vi "Restart.CacheCurrentLocation.vi"(8 "error in (no error)":errorcluster, 10 "Result":T1, 11 "State Variables":T2={"NIVS.BaseLogPath"=path "", "NIVS.SystemDefinitionFile"=path "", "NIVS.Events"={"SequenceEvent"=refnum, "SystemChangeEvent"=refnum, "WorkspaceEvent"=refnum}, "NIVS.SequenceState"=enum."Idle", "NIVS.GatewayIPAddress"="", "NIVS.DataLogSpecRef"=refnum, "NIVS.DataLogManagerRef"=refnum, "NIVS.LogSessionGUID"="", "NIVS.WorkspaceManager"=refnum, "NIVS.Deployed"=FALSE, "NIVS.ProfileRef"=refnum, "NIVS.ProfileCallback"=refnum, "NIVS.SystemStateRefs"={"CustDatRef"=refnum, "EvtRef"=refnum, "Target State User Event"=refnum}, "UI.Abort"=refnum, "UI.Pause"=refnum, "UI.EnableLogging"=refnum, "UI.Start"=refnum, "UI.LogChannels"=refnum, "UI.StartIteration"=refnum, "UI.StartStep"=refnum, "UI.Sequence"=refnum, "UI.PreviewMode"=refnum, "UI.Graph"=refnum, "UI.BaseFileName"=refnum, "UI.Profiles"=refnum, "UI.CurrentStep"=refnum, "UI.CurrentIteration"=refnum, "UI.TotalIterations"=refnum, "Sequence.AbortChannel"="", "Sequence.StepInfoChannel"="", "Sequence.Iterations"=0, "Sequence.IterationInfoChannel"="", "Sequence.#ofColumns"=0, "Events.State"=refnum, "Events.Test Result"=refnum, "Events.Progress"=refnum, "INI.Settings"={"Build Location"=path "C:/Simple Sequence Editor/SequenceRepo", "LoggingLocation"=path ""}, "UI.Skip"=refnum, "Sequence.SkipChannel"="", "Restart.Path"=path "", "UI.Duration"=refnum, "Sequence.DurationChannel"=""}) -> (0 "error out":errorcluster, 2 "Restart?":bool, 3 "State Variables out":T2={"NIVS.BaseLogPath"=path "", "NIVS.SystemDefinitionFile"=path "", "NIVS.Events"={"SequenceEvent"=refnum, "SystemChangeEvent"=refnum, "WorkspaceEvent"=refnum}, "NIVS.SequenceState"=enum."Idle", "NIVS.GatewayIPAddress"="", "NIVS.DataLogSpecRef"=refnum, "NIVS.DataLogManagerRef"=refnum, "NIVS.LogSessionGUID"="", "NIVS.WorkspaceManager"=refnum, "NIVS.Deployed"=FALSE, "NIVS.ProfileRef"=refnum, "NIVS.ProfileCallback"=refnum, "NIVS.SystemStateRefs"={"CustDatRef"=refnum, "EvtRef"=refnum, "Target State User Event"=refnum}, "UI.Abort"=refnum, "UI.Pause"=refnum, "UI.EnableLogging"=refnum, "UI.Start"=refnum, "UI.LogChannels"=refnum, "UI.StartIteration"=refnum, "UI.StartStep"=refnum, "UI.Sequence"=refnum, "UI.PreviewMode"=refnum, "UI.Graph"=refnum, "UI.BaseFileName"=refnum, "UI.Profiles"=refnum, "UI.CurrentStep"=refnum, "UI.CurrentIteration"=refnum, "UI.TotalIterations"=refnum, "Sequence.AbortChannel"="", "Sequence.StepInfoChannel"="", "Sequence.Iterations"=0, "Sequence.IterationInfoChannel"="", "Sequence.#ofColumns"=0, "Events.State"=refnum, "Events.Test Result"=refnum, "Events.Progress"=refnum, "INI.Settings"={"Build Location"=path "C:/Simple Sequence Editor/SequenceRepo", "LoggingLocation"=path ""}, "UI.Skip"=refnum, "Sequence.SkipChannel"="", "Restart.Path"=path "", "UI.Duration"=refnum, "Sequence.DurationChannel"=""})   [LabVIEW 2015, in "Simple Sequence Tools - Execution.lvlib"]
uses:
  Simple Sequence Tools - Execution.lvlib
  Types/Main.StateVariables.ctl
  Types/Execute.UserEventRefs.ctl
  <vilib>/NI Veristand/Execution/Workspace/SystemStateRegEventRef.ctl
  <vilib>/NI Veristand/Execution/Workspace/Target State Info.ctl
  <vilib>/NI Veristand/Execution/Workspace/Target State.ctl
  Types/Execution.SequenceState.ctl
  <vilib>/NI Veristand/Execution/DataLogging/DataLoggingSpecification Ref.ctl
  NationalInstruments.VeriStand.ClientAPI
  <vilib>/NI Veristand/Execution/DataLogging/IDataLogging Ref.ctl
  <vilib>/NI Veristand/Execution/Workspace/WorkspaceAPI.ctl
  NationalInstruments.VeriStand.RealTimeSequenceDefinitionApi
  <vilib>/NI Veristand/Execution/Workspace/SystemStateEventRef.ctl
  Shared/Types/INI.Settings.ctl
  Types/Results.Value.ctl
  <vilib>/NI Veristand/Execution/Workspace/NI VeriStand - Get Single Channel Value.vi
  <vilib>/NI Veristand/Execution/Workspace/NI_VS Workspace ExecutionAPI.lvlib
  <vilib>/NI Veristand/Execution/DataLogging/NI_VS Data Logging API.lvlib
  Shared/Simple Sequence Tools - Shared.lvlib
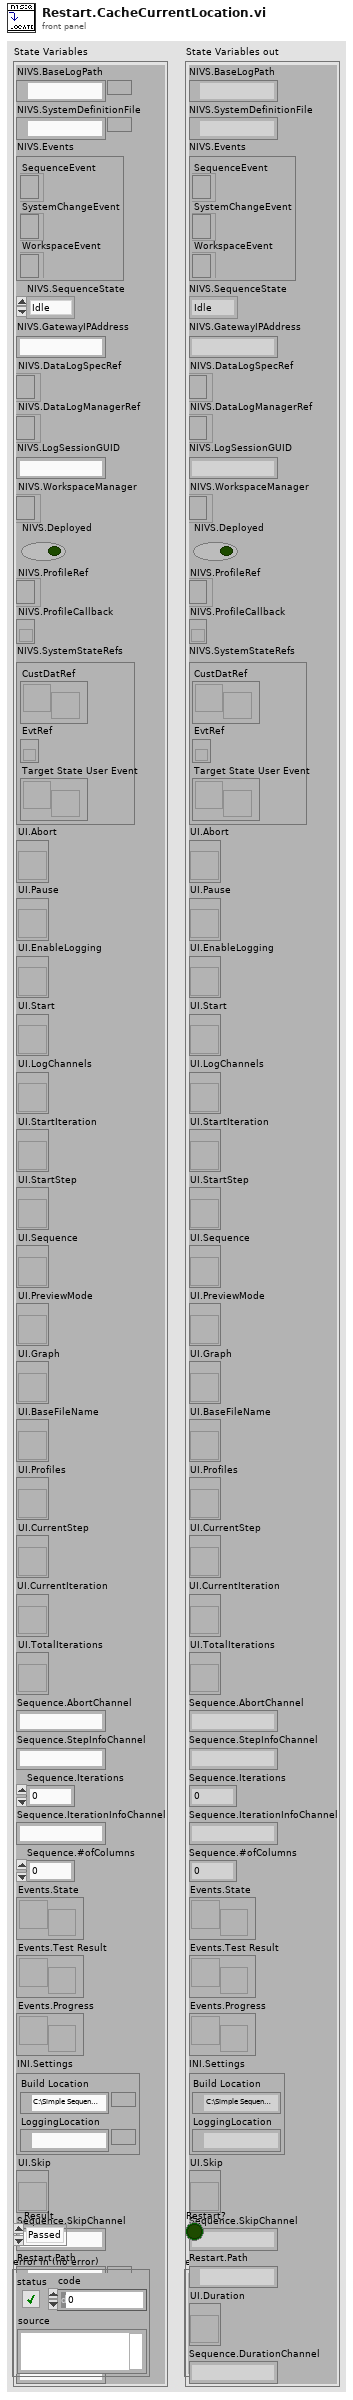
[diagram p1: front panel]
types:
  T1 = typedef "Simple Sequence Tools - Execution.lvlib/Results.Value.ctl" = enum8{"Passed", "Failed", "Aborted"}
  T2 = typedef "Simple Sequence Tools - Execution.lvlib/Main.StateVariables.ctl" = cluster{"NIVS.BaseLogPath":path, "NIVS.SystemDefinitionFile":path, "NIVS.Events":T3, "NIVS.SequenceState":T5, "NIVS.GatewayIPAddress":string, "NIVS.DataLogSpecRef":T6, "NIVS.DataLogManagerRef":T7, "NIVS.LogSessionGUID":string, "NIVS.WorkspaceManager":T8, "NIVS.Deployed":bool, "NIVS.ProfileRef":refnum<k24>, "NIVS.ProfileCallback":refnum<k27>, "NIVS.SystemStateRefs":T9, "UI.Abort":refnum<vi>, "UI.Pause":refnum<vi>, "UI.EnableLogging":refnum<vi>, "UI.Start":refnum<vi>, "UI.LogChannels":refnum<vi>, "UI.StartIteration":refnum<vi>, "UI.StartStep":refnum<vi>, "UI.Sequence":refnum<vi>, "UI.PreviewMode":refnum<vi>, "UI.Graph":refnum<vi>, "UI.BaseFileName":refnum<vi>, "UI.Profiles":refnum<vi>, "UI.CurrentStep":refnum<vi>, "UI.CurrentIteration":refnum<vi>, "UI.TotalIterations":refnum<vi>, "Sequence.AbortChannel":string, "Sequence.StepInfoChannel":string, "Sequence.Iterations":u32, "Sequence.IterationInfoChannel":string, "Sequence.#ofColumns":i32, "Events.State":refnum<user-event>, "Events.Test Result":refnum<user-event>, "Events.Progress":refnum<user-event>, "INI.Settings":T10, "UI.Skip":refnum<vi>, "Sequence.SkipChannel":string, "Restart.Path":path, "UI.Duration":refnum<vi>, "Sequence.DurationChannel":string}
  T3 = typedef "Simple Sequence Tools - Execution.lvlib/Execute.UserEventRefs.ctl" = cluster{"SequenceEvent":refnum<event-registration>, "SystemChangeEvent":T4, "WorkspaceEvent":refnum<event-registration>}
  T4 = typedef "NI_VS Workspace ExecutionAPI.lvlib/SystemStateRegEventRef.ctl" = refnum<event-registration>
  T5 = typedef "Simple Sequence Tools - Execution.lvlib/Execution.SequenceState.ctl" = enum16{"Idle", "Initializing", "Running", "Paused", "Finalizing", "Complete"}
  T6 = typedef "NI_VS Data Logging API.lvlib/DataLoggingSpecification Ref.ctl" = refnum<k24>
  T7 = typedef "NI_VS Data Logging API.lvlib/IDataLogging Ref.ctl" = refnum<k24>
  T8 = typedef "NI_VS Workspace ExecutionAPI.lvlib/WorkspaceAPI.ctl" = refnum<k24>
  T9 = typedef "NI_VS Workspace ExecutionAPI.lvlib/SystemStateEventRef.ctl" = cluster{"CustDatRef":refnum<user-event>, "EvtRef":refnum<k27>, "Target State User Event":refnum<user-event>}
  T10 = typedef "Simple Sequence Tools - Shared.lvlib/INI.Settings.ctl" = cluster{"Build Location":path, "LoggingLocation":path}
  T11 = typedef "Simple Sequence Tools - Execution.lvlib/Restart.Settings" = cluster{"LogFile":path, "Log Settings":T12[], "StimulusProfile":path, "StopIteration":u32, "StopStep":u32, "Log Channels":T16, "Base File Name":string, "Enable Logging":bool, "Profile":string, "StopDuration":dbl}
  T12 = typedef "NI_VS Data Logging API.lvlib/TDMS Channel Group.ctl" = cluster{"Group Name":string, "Group Description":string, "Group Properties":T13[], "Channels":T14[], "Time Channel Options":T15, "Time Channel Name":string}
  T13 = typedef "NI_VS Data Logging API.lvlib/TDMS Property.ctl" = cluster{"Name":string, "Value":variant}
  T14 = typedef "NI_VS Data Logging API.lvlib/TDMS Channel.ctl" = cluster{"Channel Name":string, "Channel Path":string, "Channel Description":string, "Channel Properties":T13[]}
  T15 = typedef "NI_VS Data Logging API.lvlib/Time Channel Options.ctl" = enum16{"No Time Channel", "Absolute Time", "System Time", "System Time - Microseconds", "Absolute Time as Double", "Relative To First Start Trigger", "Relative To Session Start"}
  T16 = typedef "Simple Sequence Tools - Execution.lvlib/Log.SelectedChannels.ctl" = enum16{"Channels (No System Channel)", "Aliases", "All"}
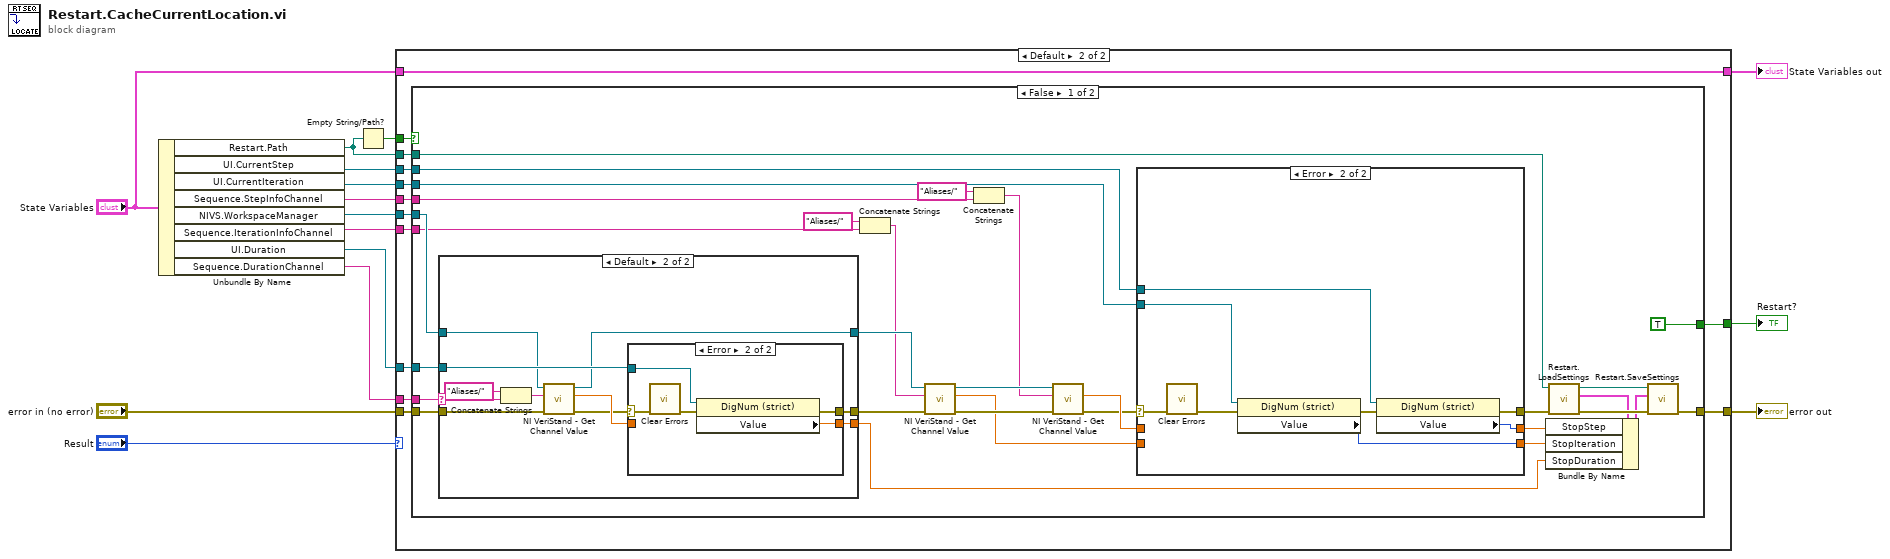
[diagram p0: block diagram]
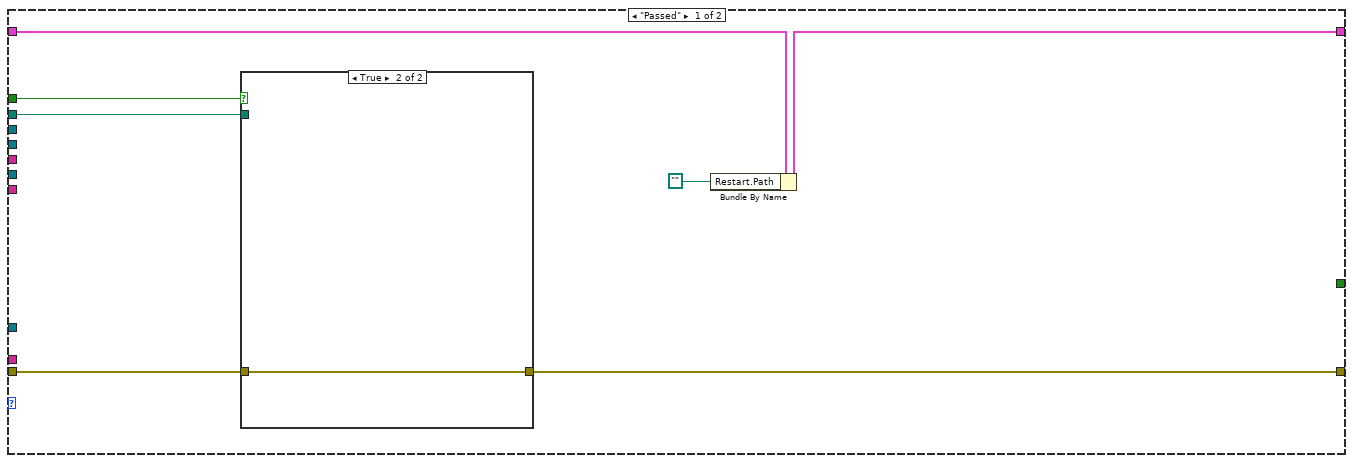
[diagram p2: hidden frame]
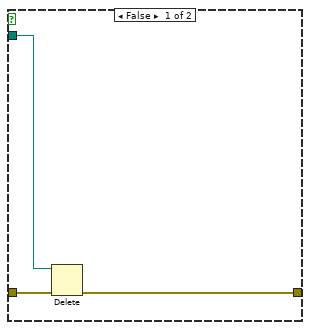
[diagram p3: hidden frame]
diagram:
  n1 = Unbundle By Name("State Variables") -> ("Restart.Path"=w6:path, "UI.CurrentStep"=w15:refnum<vi>, "UI.CurrentIteration"=w14:refnum<vi>, "Sequence.StepInfoChannel"=w7:string, "NIVS.WorkspaceManager"=w9:T8, "Sequence.IterationInfoChannel"=w8:string, "UI.Duration"=w1:refnum<vi>, "Sequence.DurationChannel"=w2:string)
  n2 = Empty String/Path?(string/path=w6) -> (empty?=w10:bool)
  n3 = case shown="Default" "Result" {
    tunnel: w10 -> [w22 w39]
    tunnel: w9 -> [_ w38]
    tunnel: w8 -> [_ w37]
    tunnel: w7 -> [_ w36]
    tunnel: w6 -> [w21 w35]
    tunnel: "error in (no error)" -> [w20 w34]
    tunnel: [w19 w33] -> w3
    tunnel: "State Variables" -> [w18 w32]
    tunnel: [w17 w32] -> w12
    tunnel: [_ w31] -> w13
    tunnel: w14 -> [_ w30]
    tunnel: w15 -> [_ w29]
    tunnel: w2 -> [_ w28]
    tunnel: w1 -> [_ w27]
    frame "Passed" {
      n4 = case shown="True" w22 {
        tunnel: w20 -> [w25 w26]
        tunnel: [w23 w26] -> w19
        tunnel: w21 -> [w24 _]
        frame False {
          n5 = Delete(path (use dialog)=w24, error in=w25) -> (error out=w23:errorcluster)  [unwired: 3 in, 2 out]
        }
        frame True {
        }
      }
      n6 = Bundle By Name(cluster=w18, "Restart.Path"=path "") -> (w17:T2)
    }
    frame Default {
      n7 = case shown="False" w39 {
        tunnel: w35 -> [w58 _]
        tunnel: w38 -> [w48 _]
        tunnel: w37 -> [w44 _]
        tunnel: w36 -> [w41 _]
        tunnel: [w60 w101] -> w33
        tunnel: w34 -> [w52 w101]
        tunnel: [TRUE _] -> w31
        tunnel: w30 -> [w54 _]
        tunnel: w29 -> [w53 _]
        tunnel: w28 -> [w50 _]
        tunnel: w27 -> [w49 _]
        frame False {
          n8 = case shown="Default" w50 {
            selector: w50 -> [_ w74]
            tunnel: w52 -> [w71 w80]
            tunnel: [w71 w79] -> w51
            tunnel: w49 -> [_ w78]
            tunnel: w48 -> [w70 w77]
            tunnel: [w70 w76] -> w47
            tunnel: [_ w75] -> w46
            frame "" {
            }
            frame Default {
              n9 = Concatenate Strings("Aliases/" ("string"), w74) -> (w73:string)
              n10 = call-poly <vilib>:"NI VeriStand - Get Channel Value.vi"("error in (no error)"=w80, "Channel"=w73, "WorkspaceManager in"=w77) -> ("error out"=w81:errorcluster, "Value"=w82:dbl, "WorkspaceManager out"=w76:T8)  [unwired: 6 in]
              n11 = case shown="Error" w81 {
                selector: w81 -> [w84 w89]
                tunnel: w82 -> [w83 _]
                tunnel: [w84 w86] -> w79
                tunnel: [w83 w85] -> w75
                tunnel: w78 -> [_ w87]
                frame No Error {
                }
                frame Error {
                  n12 = call <vilib>:"Clear Errors.vi"("error in (no error)"=w89) -> ("error out"=w88:errorcluster)  [unwired: 5 in, 1 out]
                  n13 = property class="DigNum (strict)"(reference=w87, error in=w88) -> (error out=w86:errorcluster, "Value"=w85:dbl)  [unwired: 1 out]
                }
              }
            }
          }
          n14 = Concatenate Strings("Aliases/" ("string"), w44) -> (w43:string)
          n15 = call-poly <vilib>:"NI VeriStand - Get Channel Value.vi"("error in (no error)"=w51, "Channel"=w43, "WorkspaceManager in"=w47) -> ("error out"=w68:errorcluster, "Value"=w66:dbl, "WorkspaceManager out"=w69:T8)  [unwired: 6 in]
          n16 = Concatenate Strings("Aliases/" ("string"), w41) -> (w40:string)
          n17 = call-poly <vilib>:"NI VeriStand - Get Channel Value.vi"("error in (no error)"=w68, "Channel"=w40, "WorkspaceManager in"=w69) -> ("error out"=w64:errorcluster, "Value"=w67:dbl)  [unwired: 6 in, 1 out]
          n18 = case shown="Error" w64 {
            selector: w64 -> [w92 w100]
            tunnel: w67 -> [w91 _]
            tunnel: w66 -> [w90 _]
            tunnel: [w92 w96] -> w59
            tunnel: [w91 w94] -> w56
            tunnel: [w90 w93] -> w55
            tunnel: w54 -> [_ w98]
            tunnel: w53 -> [_ w95]
            frame No Error {
            }
            frame Error {
              n19 = call <vilib>:"Clear Errors.vi"("error in (no error)"=w100) -> ("error out"=w99:errorcluster)  [unwired: 5 in, 1 out]
              n20 = property class="DigNum (strict)"(reference=w98, error in=w99) -> (error out=w97:errorcluster, "Value"=w93:u32)  [unwired: 1 out]
              n21 = property class="DigNum (strict)"(reference=w95, error in=w97) -> (error out=w96:errorcluster, "Value"=w94:u32)  [unwired: 1 out]
            }
          }
          n22 = call "Restart.LoadSettings.vi"("error in"=w59, "path (use dialog)"=w58) -> ("error out"=w63:errorcluster, "Restart Settings"=w61:T11, "path"=w57:path)  [unwired: 7 in]
          n23 = Bundle By Name(cluster=w61, "StopStep"=w56, "StopIteration"=w55, "StopDuration"=w46) -> (w62:T11)
          n24 = call "Restart.SaveSettings.vi"("error in"=w63, "Restart Settings"=w62, "datalog path (use dialog)"=w57) -> ("error out"=w60:errorcluster)  [unwired: 7 in, 1 out]
        }
        frame True {
        }
      }
    }
  }
  "error out" <- w3
  "State Variables out" <- w12
  "Restart?" <- w13
